vi "Performance Test.vi"() -> ()   [LabVIEW 2021]
uses:
  typedef/Topic Full Names.ctl
  <vilib>/Platform/TimedLoop/XDataNode/timing_clust.ctl
  <vilib>/Platform/TimedLoop/XDataNode/nitl_modes.ctl
  <vilib>/Platform/TimedLoop/XDataNode/wakeup.ctl
  1d7c6f29-a82a-4c55-90c2-8d5dc10d4cfc.vi
  17fd5a01-9941-4072-bead-c11bfc9bccae.vi
  ed299c19-1de2-4aef-bebd-b48bd10f6d98.vi
  968a0517-1209-4268-883c-89309fdc9691.vi
  d644dcab-1457-4dd0-b19b-55e0bc57f857.vi
  a6d30745-cc28-47f9-89da-0309ddd02839.vi
  ca39f006-b041-4da7-9f13-a82cb085cbb3.vi
  5bfc589c-c630-4e63-a8b4-f54732edfa77.vi
  394fcb2d-213c-4a5d-8836-742277111c33.vi
  47ad3e17-e753-4109-9264-7bc845309f70.vi
  34d71a64-62ff-4078-a387-3a58d5c35b2e.vi
  5417b091-9016-444e-b18d-e7968ccf46ca.vi
  17355536-f9ad-45df-8cdf-a653dafc3748.vi
  31a05237-38ce-4d36-92b2-ec91211d35c9.vi
  29b1b57c-db52-4db6-85d2-2783ba32f171.vi
  8285cac4-4baf-4ff9-aee7-9ff83ddf547c.vi
  d69192ad-9d02-4c06-9baa-091e86991072.vi
  801e2a67-ee41-44d4-a069-6c7db1e2d5be.vi
  84590647-50eb-4c0b-b77c-fbe9ef827284.vi
  20063719-1bf0-46dd-9a55-ff35ed26eb0a.vi
  38f10348-bd34-475b-a8eb-5ab5d485f78a.vi
  b3b3740b-c499-4e36-8042-ad8fb7248740.vi
  a2b9d25c-82f9-44a5-b179-014c788887ad.vi
  60e7bcfe-7ed0-4ed5-a910-62fb5c100d45.vi
  8a134818-91b4-4009-8209-aee668485e20.vi
  150ac17d-bb1a-4f1c-be46-9412ac39043d.vi
  1faeae08-4a57-41f3-9a76-3e5847141804.vi
  SubVIs/Get Path.vi
  SubVIs/Convert Error.vi
  1d7c6f29-a82a-4c55-90c2-8d5dc10d4cfc.vi/f164bb55-fadc-406a-97d8-e3295a396b46.vi
  SubVIs/Add Error.vi
  Refnum/BB from Refnum.vi
  Refnum/BB Writer to Refnum.vi
  <vilib>/CIF Foundation/CIF Utilities/File/File/File Not Found Error Update.vi
  17fd5a01-9941-4072-bead-c11bfc9bccae.vi/15451e88-64ef-462d-9cc0-58968935b893.vi
  Refnum/BB Reader to Refnum.vi
  Refnum/BB Writer from Refnum.vi
  Refnum/BB Reader from Refnum.vi
  5bfc589c-c630-4e63-a8b4-f54732edfa77.vi/f164bb55-fadc-406a-97d8-e3295a396b46.vi
  394fcb2d-213c-4a5d-8836-742277111c33.vi/15451e88-64ef-462d-9cc0-58968935b893.vi
  31a05237-38ce-4d36-92b2-ec91211d35c9.vi/f164bb55-fadc-406a-97d8-e3295a396b46.vi
  29b1b57c-db52-4db6-85d2-2783ba32f171.vi/15451e88-64ef-462d-9cc0-58968935b893.vi
  20063719-1bf0-46dd-9a55-ff35ed26eb0a.vi/3bd89bd1-b605-4b55-aa60-227046f12b11.vi
  38f10348-bd34-475b-a8eb-5ab5d485f78a.vi/bd005753-9160-49ee-ba23-7aa8055d86ff.vi
  Refnum/BB Raw Writer to Refnum.vi
  Refnum/BB Raw Reader to Refnum.vi
  Refnum/BB Raw Reader from Refnum.vi
  Refnum/BB Raw Writer from Refnum.vi
  <vilib>/Utility/error.llb/Trim Whitespace.vi
  SubVIs/Add Error Core.vi
  <vilib>/CIF Foundation/CIF Utilities/DataTypes/Utilities/Get Element Info of Variant.vi
  SubVIs/Get Type String.vi
  <vilib>/CIF Foundation/CIF Utilities/DataTypes/Utilities/Get JSON Descriptor of Variant.vi
  SubVIs/Convert Error Core.vi
  <vilib>/CIF Foundation/CIF Utilities/File/SubVIs/File Not Found Error Core.vi
  <vilib>/Platform/TimedLoop/XDataNode/XDataNode.xnode
  <vilib>/Platform/TimedLoop/XDataNode/XDNodeRunTimeDep.lvlib
  Iceoryx.lvlib
panel:
  out "avg read raw large array":dbl
  out "max read raw large array":dbl
  out "avg read large array":dbl
  out "max read large array":dbl
  out "avg write double":dbl
  out "max write double":dbl
  out "avg read double no writer":dbl
  out "max read double no writer":dbl
  in  "stop":bool
  out "avg read double":dbl
  out "max read double":dbl
  out "pass":bool
  out "error out":errorcluster
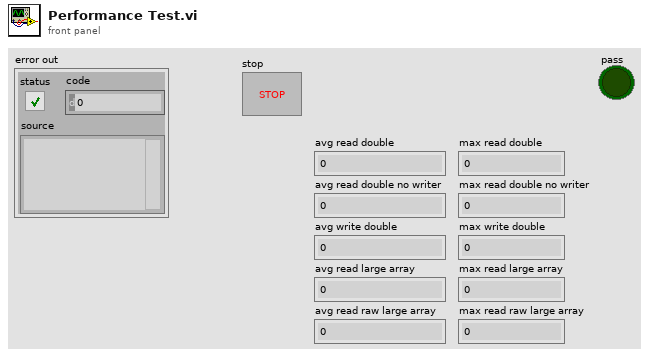
[diagram p1: front panel]
types:
  T1 = typedef "Iceoryx.lvlib/Topic Full Names.ctl" = cluster{"BlackBoard":string, "Topic":string, "Type Override":string}
  T2 = typedef "XDNodeRunTimeDep.lvlib/timing_clust.ctl" = cluster{"Expected End [f-1]":u64, "Actual End [f-1]":u64, "Finished Late? [f-1]":bool, "Expected End [i-1]":u64, "Actual End [i-1]":u64, "Finished Late? [i-1]":bool, "Expected Start [i]":u64, "Actual Start [i]":u64, "Expected Start [f]":u64, "Actual Start [f]":u64, "Source Name":string, "Structure Name":string, "Period":i64, "Deadline":i64, "Offset":i64, "Start":i64, "Priority":i32, "Timeout":i32, "Mode":T3, "Wakeup Reason":T4, "Error":errorcluster, "Source Type":string, "Secondary Source Type":string, "Global End Time":u64, "Global Start Time":u64, "Frame Duration":u64, "Iteration Duration":u64, "Assigned CPU":i32, "I/O Scan Engine Mode":u32}
  T3 = typedef "XDNodeRunTimeDep.lvlib/nitl_modes.ctl" = enum32{"No Change", "Process missed periods, maintain original phase", "Discard missed periods, maintain original phase", "Process missed periods, ignore original phase", "Discard missed periods, ignore original phase"}
  T4 = typedef "XDNodeRunTimeDep.lvlib/wakeup.ctl" = enum32{"Normal", "Aborted", "Asynchronous wakeup", "Timing source error", "Timed loop error", "Timeout"}
  T5 = typedef "Iceoryx.lvlib/BB Refnum.ctl" = cluster{"refnum":u64, "BB":enum8{"bb"}}
  T6 = typedef "Iceoryx.lvlib/BB Writer Refnum.ctl" = cluster{"refnum":u64, "BB Writer":enum8{"bb_writer"}}
  T7 = typedef "Iceoryx.lvlib/BB Reader Refnum.ctl" = cluster{"refnum":u64, "BB Reader":enum8{"bb_reader"}}
  T8 = typedef "Iceoryx.lvlib/BB Raw Writer Refnum.ctl" = cluster{"refnum":u64, "BB Raw Writer":enum8{"bb_raw_writer"}}
  T9 = typedef "Iceoryx.lvlib/BB Raw Reader Refnum.ctl" = cluster{"refnum":u64, "BB Raw Reader":enum8{"bb_raw_reader"}}
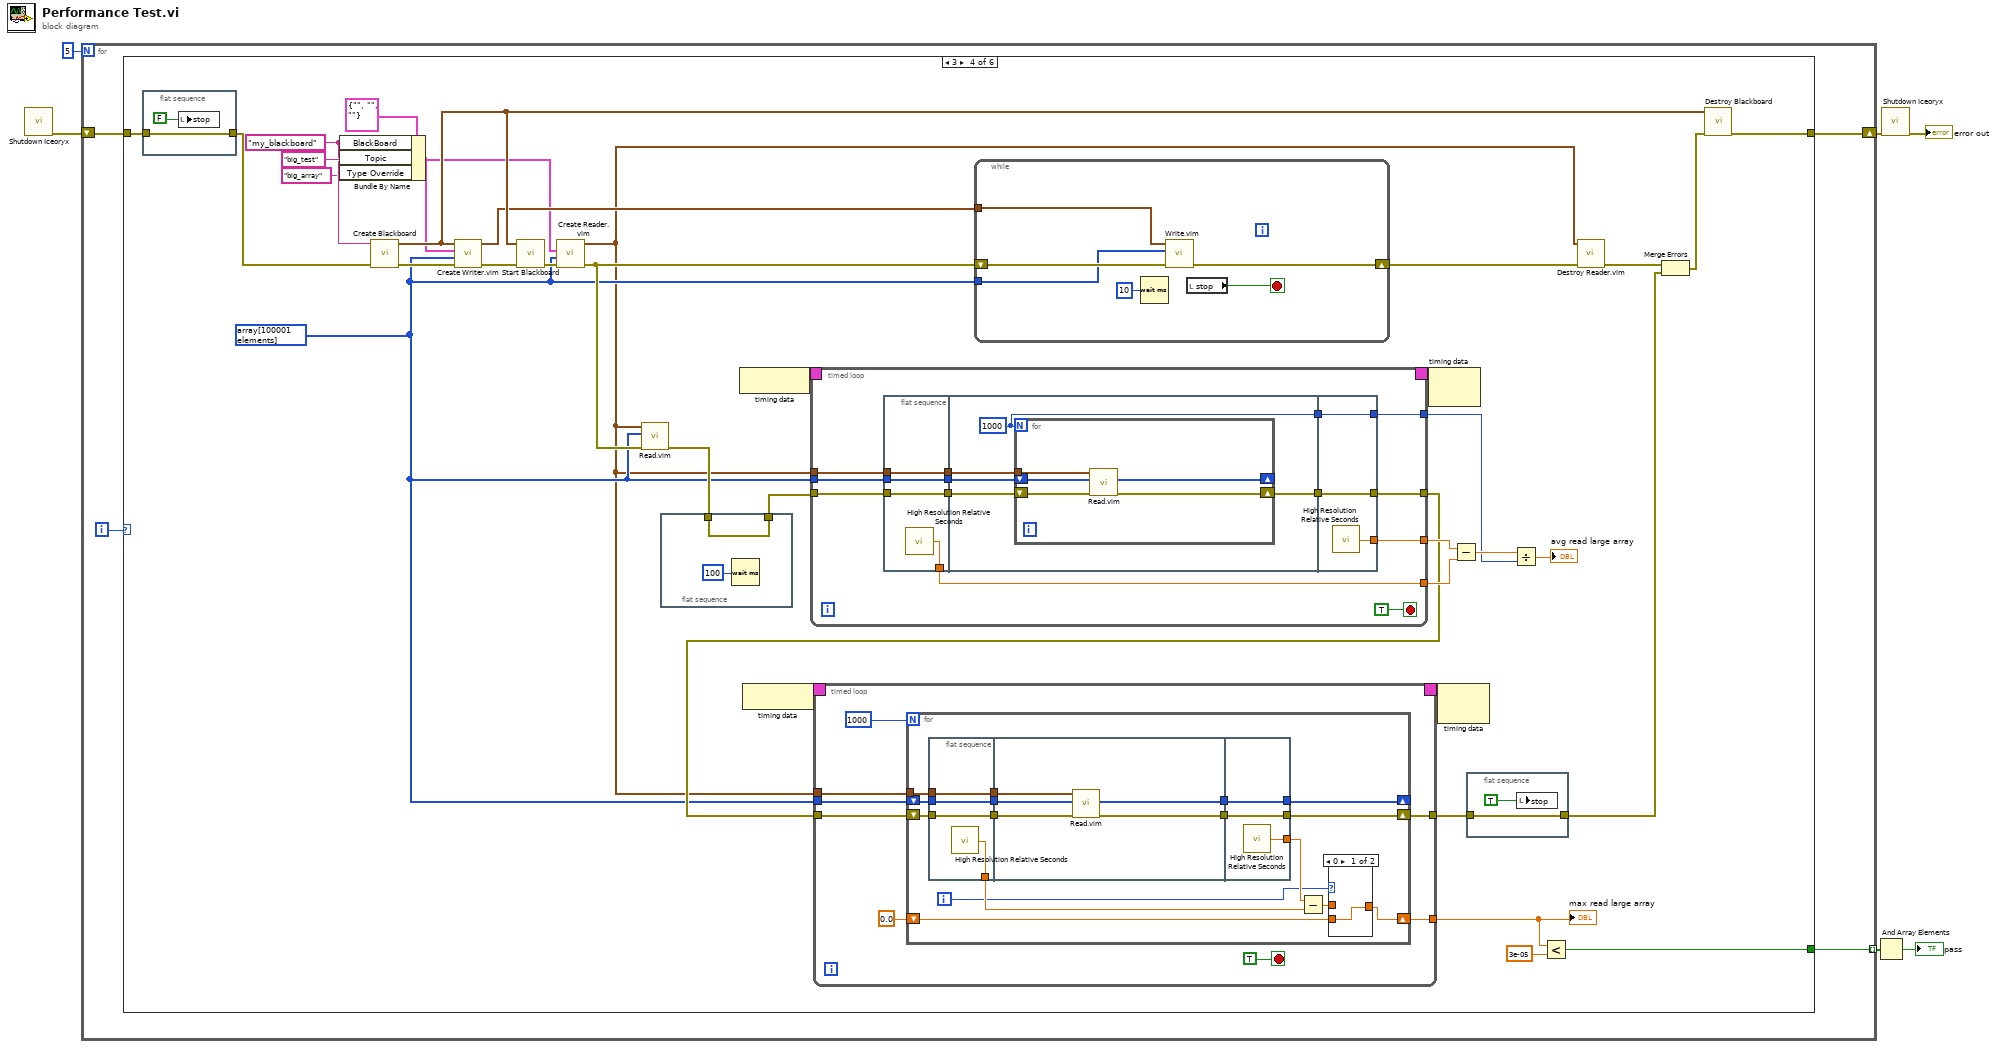
[diagram p0: block diagram]
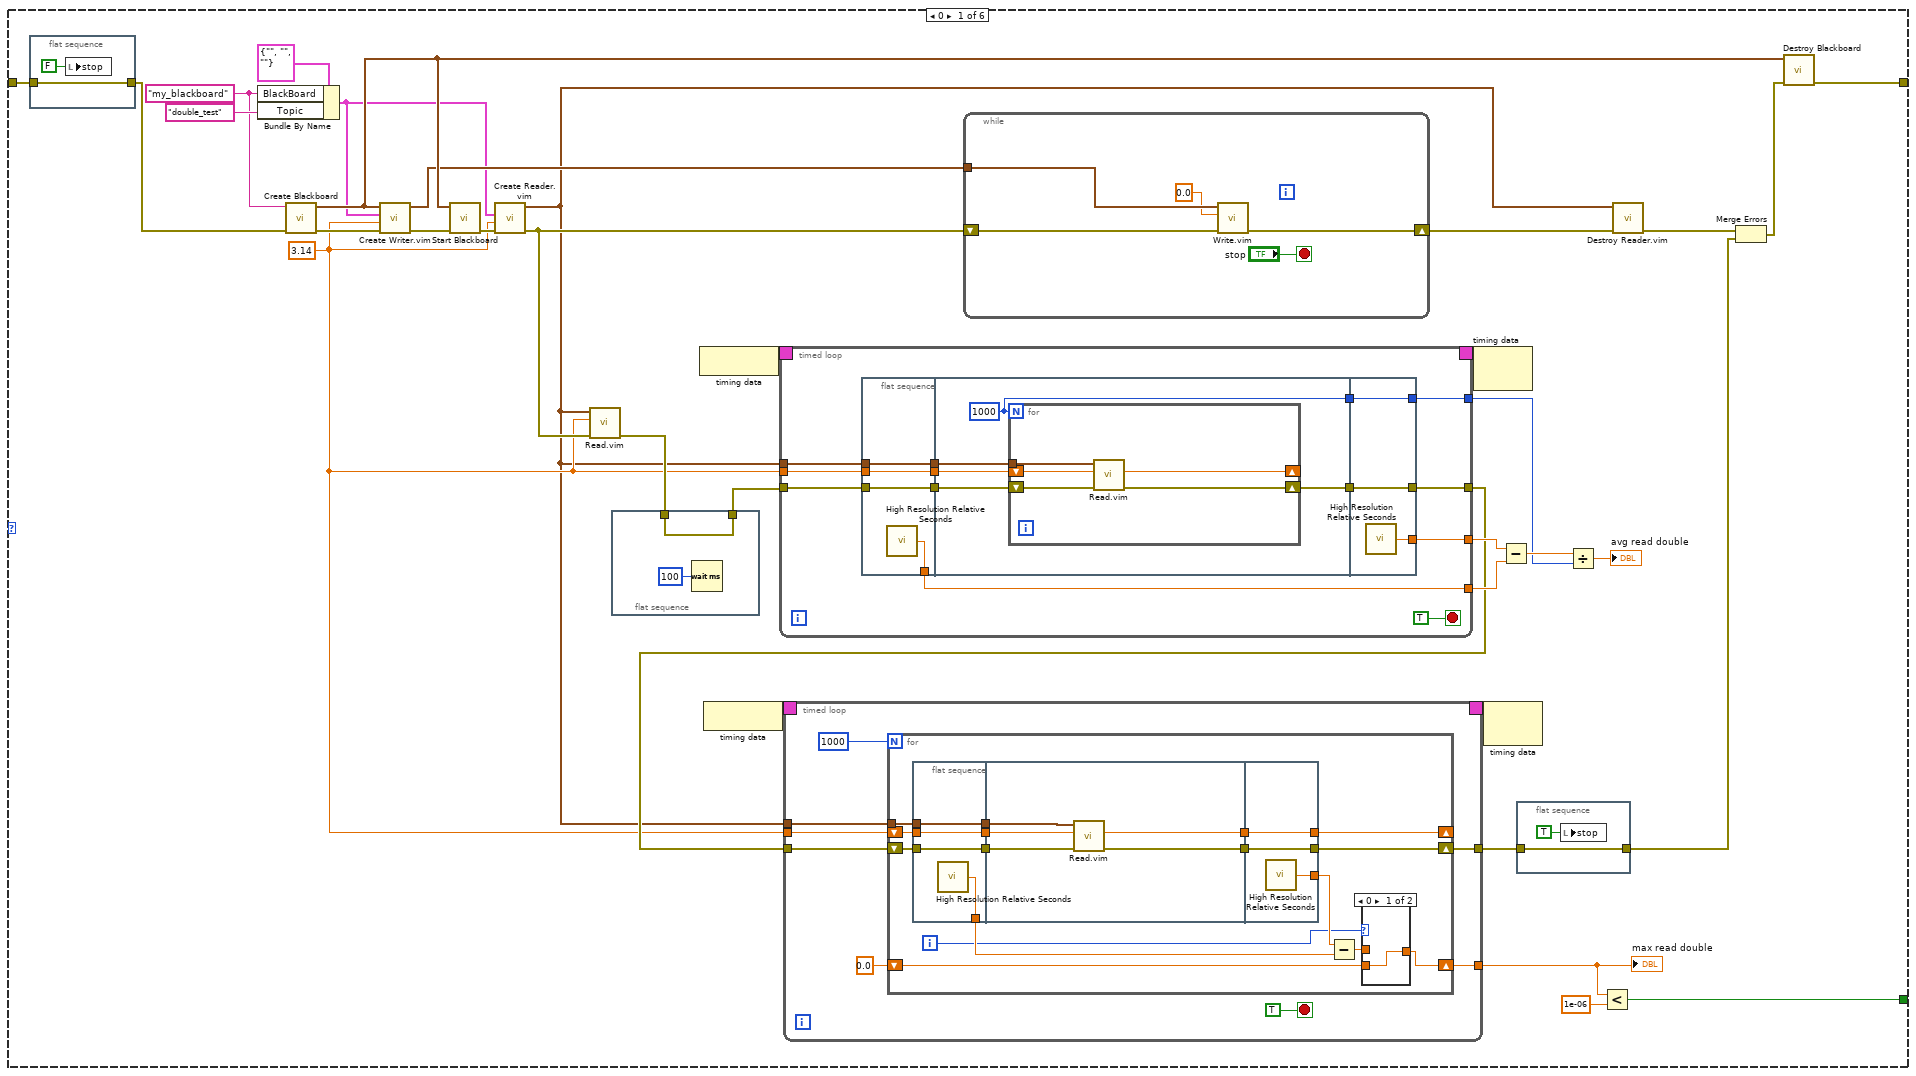
[diagram p2: hidden frame]
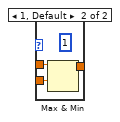
[diagram p3: hidden frame]
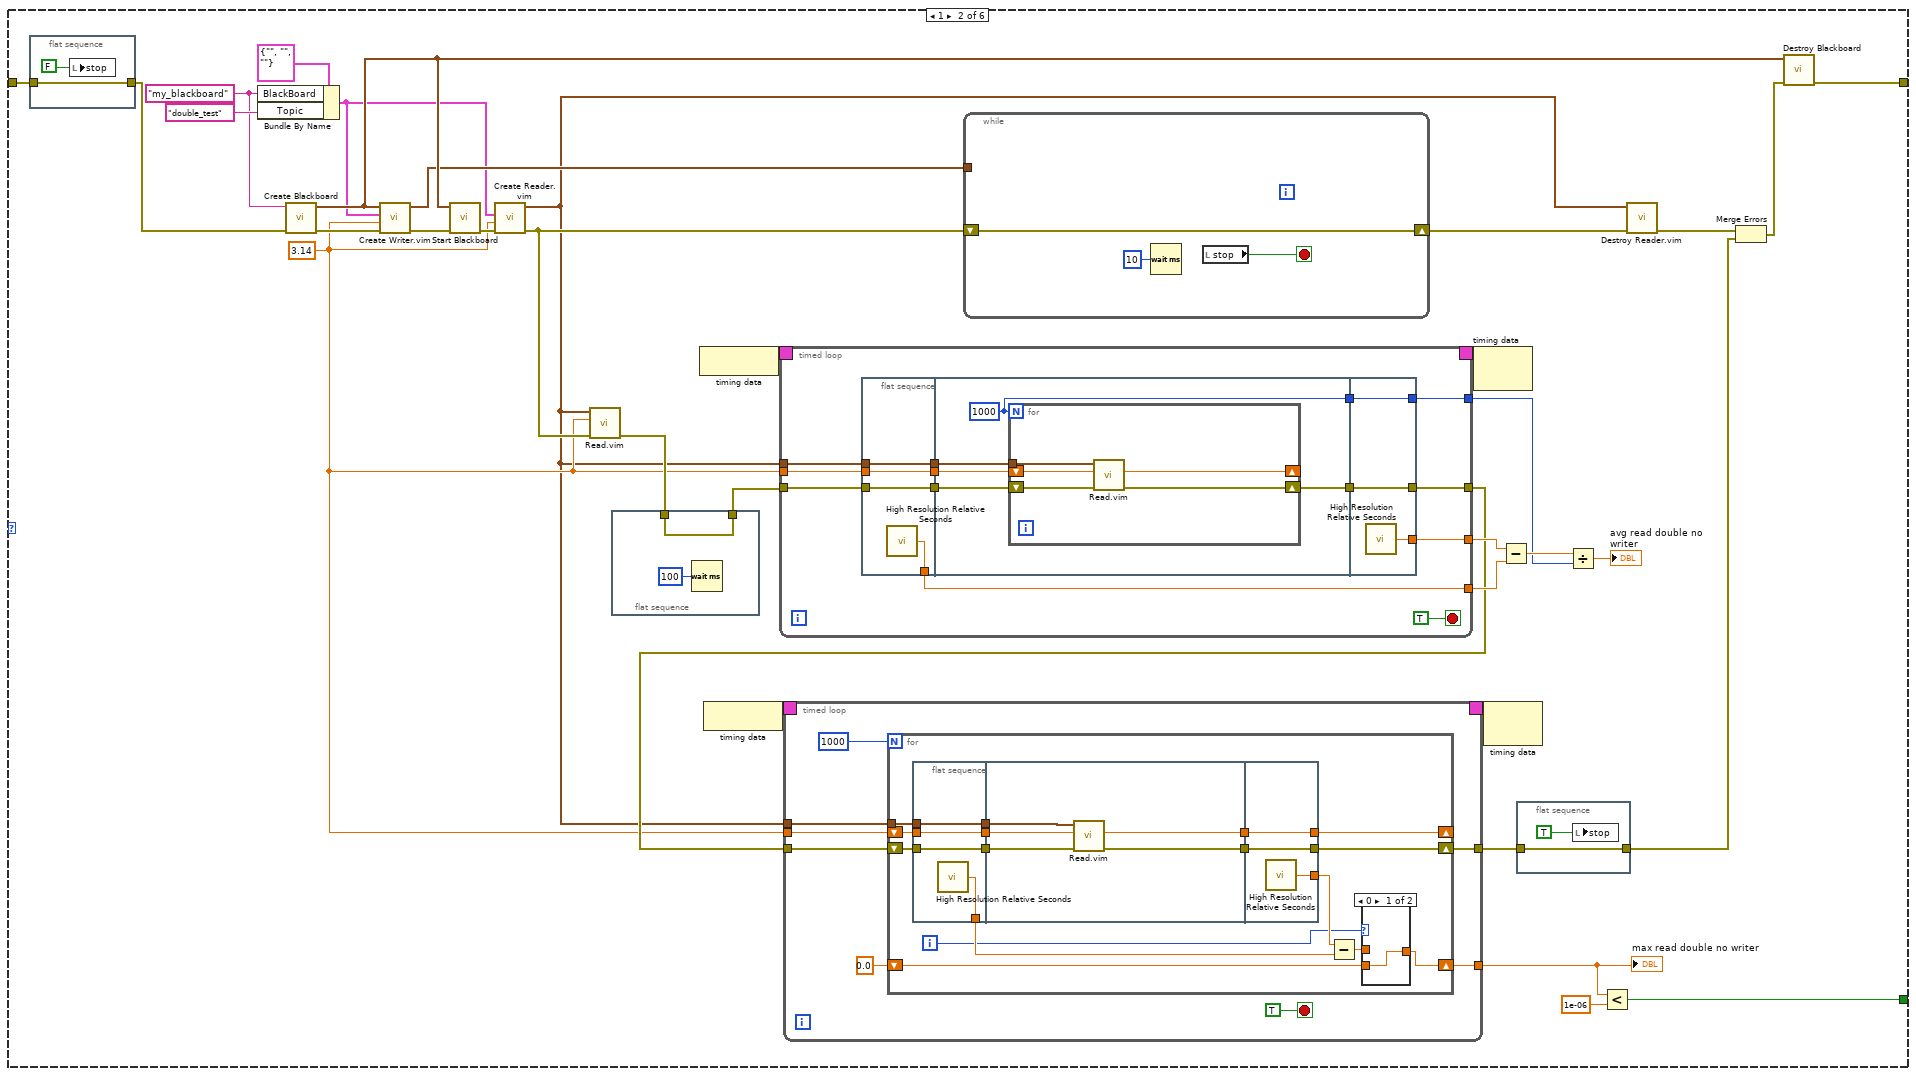
[diagram p4: hidden frame]
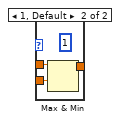
[diagram p5: hidden frame]
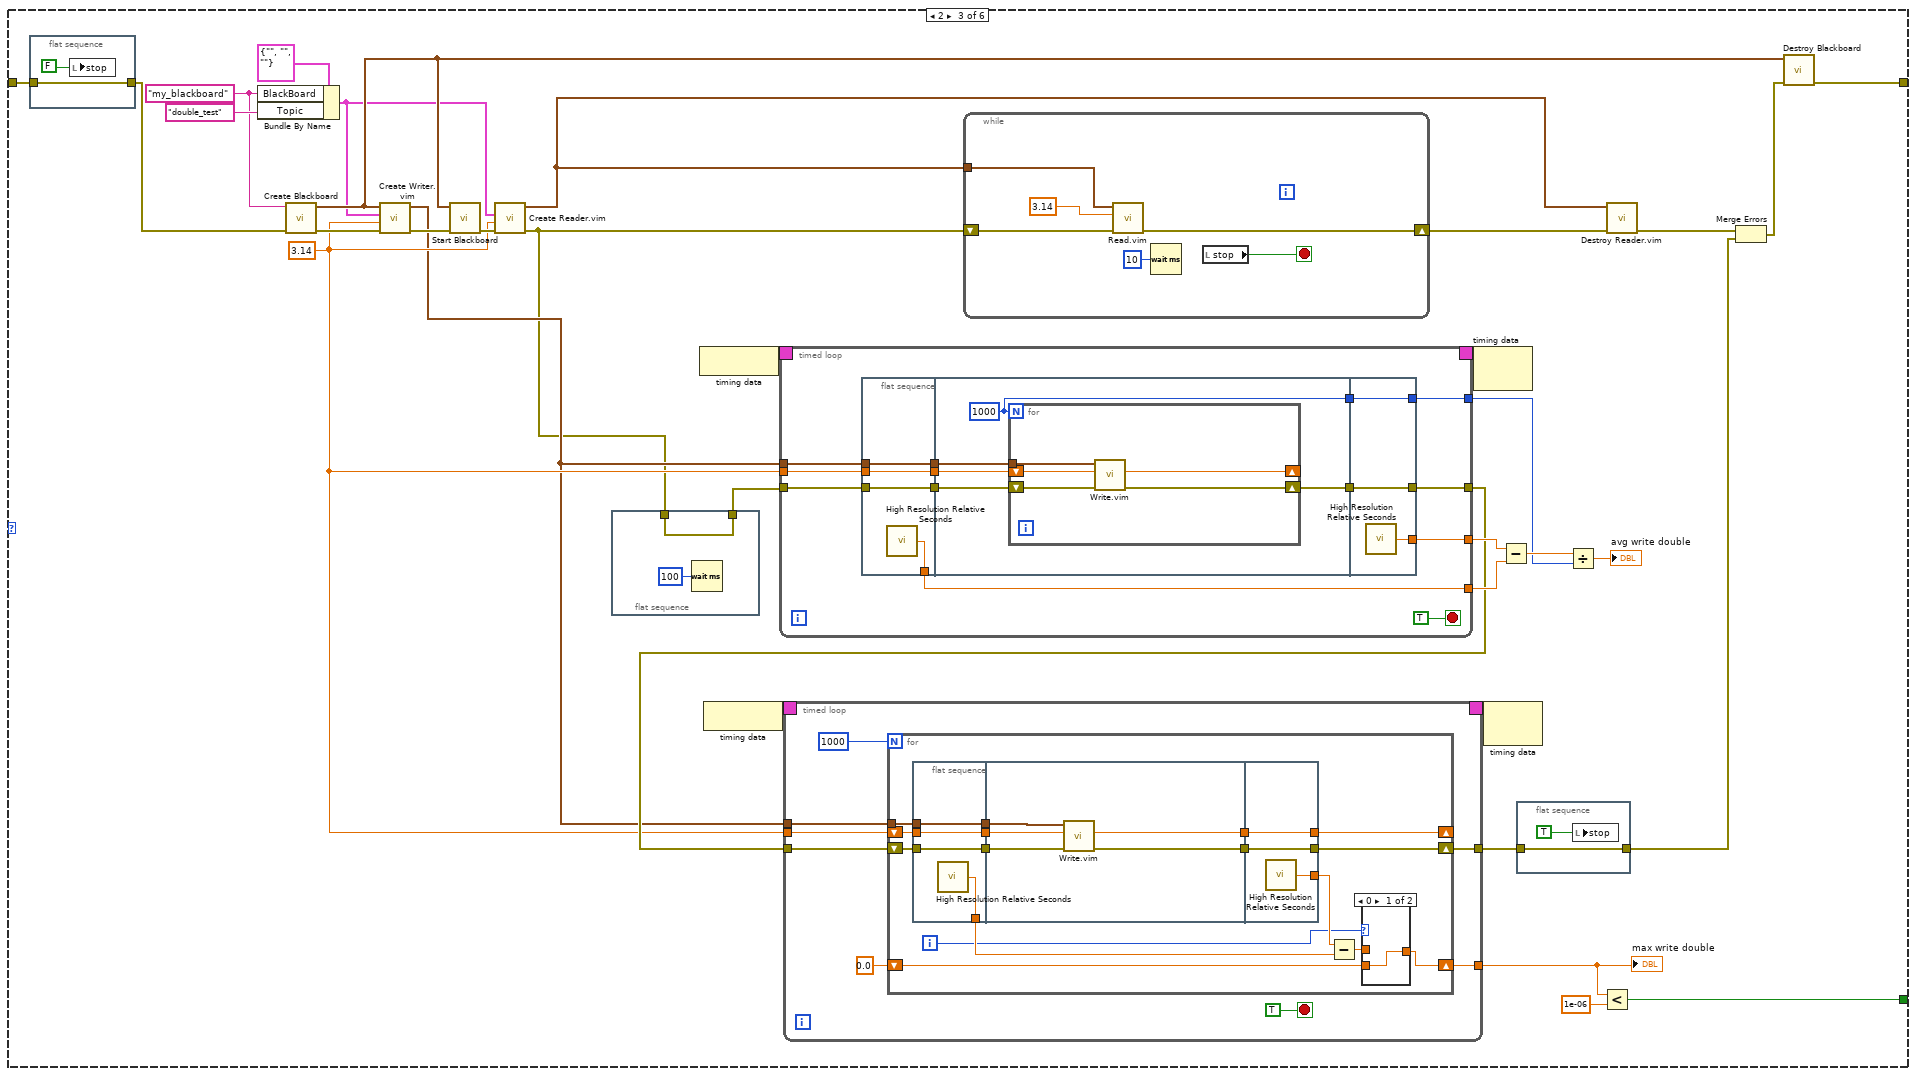
[diagram p6: hidden frame]
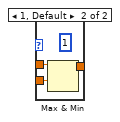
[diagram p7: hidden frame]
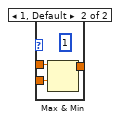
[diagram p8: hidden frame]
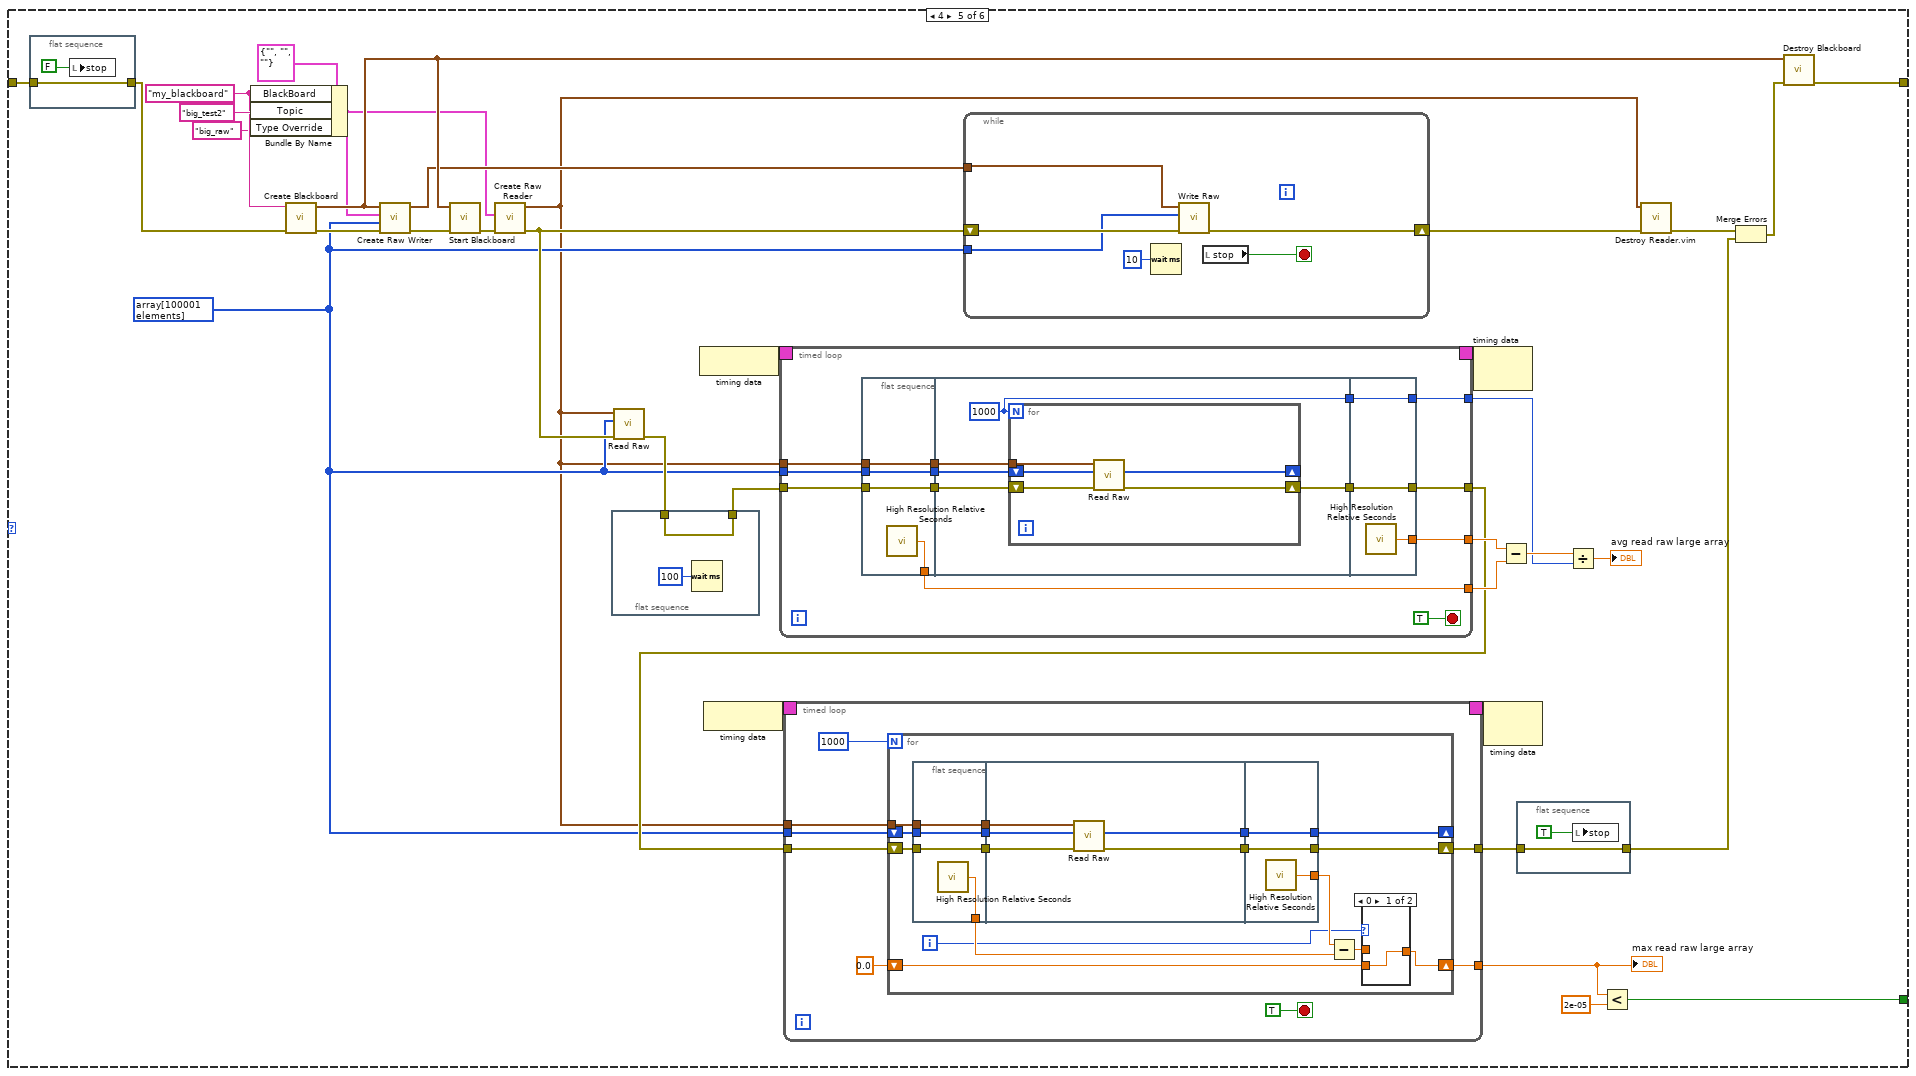
[diagram p9: hidden frame]
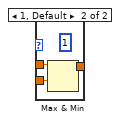
[diagram p10: hidden frame]
diagram:
  n1 = call "Shutdown Iceoryx.vi"() -> ("error out"=w4:errorcluster)  [unwired: 11 in]
  n2 = for {
    N: 5 -> [_]
    tunnel: [w10] -> w2 mode=indexing
    shift-right: [w9] -> w6
    shift-left: w4 -> [w8]
    i -> [w7]
    n3 = case shown="3" w7 {
      tunnel: [w31 w155 w276 w402 w528 _] -> w10
      tunnel: [w26 w150 w271 w397 w523 w633] -> w9
      tunnel: w8 -> [w15 w139 w263 w387 w515 w633]
      frame 0 {
        w19 = "my_blackboard" ("Blackboard name")
        w18 = 3.14 ("Data")
        n4 = flat-sequence {
          tunnel: w15 -> [w52]
          tunnel: [w52] -> w14
          frame #0 {
            n5 = local write "stop"(FALSE ("stop")) -> ()
          }
        }
        n6 = Bundle By Name(cluster=T1 {"BlackBoard"="", "Topic"="", "Type Override"=""} ("Topic Full Names"), "BlackBoard"=w19, "Topic"="double_test" ("topic")) -> (w20:T1)
        n7 = call "Create Blackboard.vi"("error in (no error)"=w14, "Blackboard name"=w19) -> ("error out"=w30:errorcluster, "Blackboard Reference"=w28:T5)  [unwired: 8 in]
        n8 = call "Create Writer.vim"("error in (no error)"=w30, "Data"=w18, "Topic Name"=w20, "BlackBoard Reference"=w28) -> ("error out"=w29:errorcluster, "Writer Reference"=w25:T6)  [unwired: 5 in, 1 out]
        n9 = call "Start Blackboard.vi"("error in (no error)"=w29, "Blackboard Reference"=w28) -> ("error out"=w27:errorcluster)  [unwired: 9 in]
        n10 = call "Create Reader.vim"("error in (no error)"=w27, "Data Type"=w18, "Topic Name"=w20) -> ("error out"=w24:errorcluster, "Reader Reference"=w11:T7)  [unwired: 6 in, 1 out]
        n11 = call "Read.vim"("error in (no error)"=w24, "Data In"=w18, "Reader Reference"=w11) -> ("error out"=w23:errorcluster)  [unwired: 6 in, 2 out]
        n12 = flat-sequence {
          tunnel: w23 -> [w56]
          tunnel: [w56] -> w33
          frame #0 {
            n13 = Wait (ms)(milliseconds to wait=u32 100) -> ()  [unwired: 1 out]
          }
        }
        n14 = node-c288() -> (w45:T2)
        n15 = node-c288() -> (w43:T2)
        n16 = timed-loop {
          timing: w45 -> [_]
          timing-out: [_] -> w44
          tunnel: w11 -> [w103]
          tunnel: w33 -> [w113]
          tunnel: [w110] -> w37
          tunnel: [w108] -> w41
          tunnel: [w107] -> w40
          tunnel: [w106] -> w38
          tunnel: w18 -> [w101]
          stop <- TRUE stop-if-true
          n17 = flat-sequence {
            tunnel: w113 -> [w117]
            tunnel: [w117] -> w111
            tunnel: [w116] -> w107
            tunnel: [w115] -> w104
            tunnel: w103 -> [w115]
            tunnel: [w114] -> w102
            tunnel: w101 -> [w114]
            tunnel: w111 -> [w122]
            tunnel: [w121] -> w109
            tunnel: [w120] -> w105
            tunnel: w104 -> [w119]
            tunnel: w102 -> [w118]
            tunnel: [w130] -> w110
            tunnel: w109 -> [w130]
            tunnel: [w129] -> w108
            tunnel: [w128] -> w106
            tunnel: w105 -> [w128]
            frame #0 {
              n18 = call <vilib>:"High Resolution Relative Seconds.vi"() -> ("relative seconds"=w116:dbl)
            }
            frame #1 {
              w120 = 1000
              n19 = for {
                N: w120 -> [_]
                shift-right: [w124] -> _
                shift-left: w118 -> [w123]
                shift-right: [w125] -> w121
                shift-left: w122 -> [w126]
                tunnel: w119 -> [w127]
                n20 = call "Read.vim"("error in (no error)"=w126, "Data In"=w123, "Reader Reference"=w127) -> ("error out"=w125:errorcluster, "Data Out"=w124:dbl)  [unwired: 6 in, 1 out]
              }
            }
            frame #2 {
              n21 = call <vilib>:"High Resolution Relative Seconds.vi"() -> ("relative seconds"=w129:dbl)
            }
          }
        }
        n22 = timed-loop {
          timing: w43 -> [_]
          timing-out: [_] -> w42
          tunnel: w37 -> [w64]
          tunnel: [w62] -> w32
          tunnel: [w59] -> w35
          tunnel: w18 -> [w58]
          tunnel: w11 -> [w57]
          stop <- TRUE stop-if-true
          n23 = for {
            N: 1000 -> [_]
            shift-right: [w75] -> _
            shift-left: w58 -> [w77]
            shift-right: [w74] -> w62
            shift-left: w64 -> [w76]
            shift-right: [w69] -> w59
            shift-left: 0.0 -> [w70]
            tunnel: w57 -> [w65]
            i -> [w68]
            n24 = flat-sequence {
              tunnel: w76 -> [w87]
              tunnel: w77 -> [w88]
              tunnel: [w88] -> w80
              tunnel: [w87] -> w79
              tunnel: [w86] -> w72
              tunnel: [w85] -> w66
              tunnel: w65 -> [w85]
              tunnel: w80 -> [w89]
              tunnel: w79 -> [w93]
              tunnel: [w91] -> w78
              tunnel: [w90] -> w67
              tunnel: w66 -> [w92]
              tunnel: [w96] -> w75
              tunnel: w78 -> [w96]
              tunnel: [w95] -> w74
              tunnel: [w94] -> w73
              tunnel: w67 -> [w95]
              frame #0 {
                n25 = call <vilib>:"High Resolution Relative Seconds.vi"() -> ("relative seconds"=w86:dbl)
              }
              frame #1 {
                n26 = call "Read.vim"("error in (no error)"=w93, "Data In"=w89, "Reader Reference"=w92) -> ("error out"=w90:errorcluster, "Data Out"=w91:dbl)  [unwired: 6 in, 1 out]
              }
              frame #2 {
                n27 = call <vilib>:"High Resolution Relative Seconds.vi"() -> ("relative seconds"=w94:dbl)
              }
            }
            n28 = Subtract(x=w73, y=w72) -> (x-y=w71:dbl)
            n29 = case shown="0" w68 {
              tunnel: w71 -> [_ w84]
              tunnel: w70 -> [w81 w83]
              tunnel: [w81 w82] -> w69
              frame 0 {
              }
              frame 1, Default {
                (unwired) u32 1 ("milliseconds to wait")
                n30 = Max & Min(x=w84, y=w83) -> (max(x,y)=w82:dbl)  [unwired: 1 out]
              }
            }
          }
        }
        "max read double" <- w35
        n31 = while {
          shift-right: [w47] -> w13
          shift-left: w24 -> [w48]
          tunnel: w25 -> [w49]
          stop <- "stop" stop-if-true
          n32 = call "Write.vim"("error in (no error)"=w48, "Data In"=0.0, "Writer Reference"=w49) -> ("error out"=w47:errorcluster)  [unwired: 7 in, 1 out]
        }
        n33 = node-c288(w44) -> ()  [unwired: 1 out]
        n34 = node-c288(w42) -> ()  [unwired: 1 out]
        n35 = Subtract(x=w41, y=w40) -> (x-y=w39:dbl)
        n36 = flat-sequence {
          tunnel: w32 -> [w54]
          tunnel: [w54] -> w17
          frame #0 {
            n37 = local write "stop"(TRUE ("stop")) -> ()
          }
        }
        n38 = Divide(x=w39, y=w38) -> (x/y=→"avg read double":dbl)
        n39 = Less?(x=w35, y=1e-06) -> (x < y?=w31:bool)
        n40 = call "Destroy Reader.vim"("error in (no error)"=w13, "Reader Reference"=w11) -> ("error out"=w12:errorcluster)  [unwired: 9 in]
        n41 = Merge Errors(w12, w17) -> (w16:errorcluster)
        n42 = call "Destroy Blackboard.vi"("error in (no error)"=w16, "Blackboard Reference"=w28) -> ("error out"=w26:errorcluster)  [unwired: 8 in, 1 out]
      }
      frame 1 {
        w143 = "my_blackboard" ("Blackboard name")
        w142 = 3.14 ("Data")
        n43 = flat-sequence {
          tunnel: w139 -> [w174]
          tunnel: [w174] -> w138
          frame #0 {
            n44 = local write "stop"(FALSE ("stop")) -> ()
          }
        }
        n45 = Bundle By Name(cluster=T1 {"BlackBoard"="", "Topic"="", "Type Override"=""} ("Topic Full Names"), "BlackBoard"=w143, "Topic"="double_test" ("topic")) -> (w144:T1)
        n46 = call "Create Blackboard.vi"("error in (no error)"=w138, "Blackboard name"=w143) -> ("error out"=w154:errorcluster, "Blackboard Reference"=w152:T5)  [unwired: 8 in]
        n47 = call "Create Writer.vim"("error in (no error)"=w154, "Data"=w142, "Topic Name"=w144, "BlackBoard Reference"=w152) -> ("error out"=w153:errorcluster, "Writer Reference"=w149:T6)  [unwired: 5 in, 1 out]
        n48 = call "Start Blackboard.vi"("error in (no error)"=w153, "Blackboard Reference"=w152) -> ("error out"=w151:errorcluster)  [unwired: 9 in]
        n49 = call "Create Reader.vim"("error in (no error)"=w151, "Data Type"=w142, "Topic Name"=w144) -> ("error out"=w148:errorcluster, "Reader Reference"=w135:T7)  [unwired: 6 in, 1 out]
        n50 = call "Read.vim"("error in (no error)"=w148, "Data In"=w142, "Reader Reference"=w135) -> ("error out"=w147:errorcluster)  [unwired: 6 in, 2 out]
        n51 = flat-sequence {
          tunnel: w147 -> [w178]
          tunnel: [w178] -> w157
          frame #0 {
            n52 = Wait (ms)(milliseconds to wait=u32 100) -> ()  [unwired: 1 out]
          }
        }
        n53 = node-c288() -> (w169:T2)
        n54 = node-c288() -> (w167:T2)
        n55 = timed-loop {
          timing: w169 -> [_]
          timing-out: [_] -> w168
          tunnel: w135 -> [w225]
          tunnel: w157 -> [w235]
          tunnel: [w232] -> w161
          tunnel: [w230] -> w165
          tunnel: [w229] -> w164
          tunnel: [w228] -> w162
          tunnel: w142 -> [w223]
          stop <- TRUE stop-if-true
          n56 = flat-sequence {
            tunnel: w235 -> [w239]
            tunnel: [w239] -> w233
            tunnel: [w238] -> w229
            tunnel: [w237] -> w226
            tunnel: w225 -> [w237]
            tunnel: [w236] -> w224
            tunnel: w223 -> [w236]
            tunnel: w233 -> [w244]
            tunnel: [w243] -> w231
            tunnel: [w242] -> w227
            tunnel: w226 -> [w241]
            tunnel: w224 -> [w240]
            tunnel: [w252] -> w232
            tunnel: w231 -> [w252]
            tunnel: [w251] -> w230
            tunnel: [w250] -> w228
            tunnel: w227 -> [w250]
            frame #0 {
              n57 = call <vilib>:"High Resolution Relative Seconds.vi"() -> ("relative seconds"=w238:dbl)
            }
            frame #1 {
              w242 = 1000
              n58 = for {
                N: w242 -> [_]
                shift-right: [w246] -> _
                shift-left: w240 -> [w245]
                shift-right: [w247] -> w243
                shift-left: w244 -> [w248]
                tunnel: w241 -> [w249]
                n59 = call "Read.vim"("error in (no error)"=w248, "Data In"=w245, "Reader Reference"=w249) -> ("error out"=w247:errorcluster, "Data Out"=w246:dbl)  [unwired: 6 in, 1 out]
              }
            }
            frame #2 {
              n60 = call <vilib>:"High Resolution Relative Seconds.vi"() -> ("relative seconds"=w251:dbl)
            }
          }
        }
        n61 = timed-loop {
          timing: w167 -> [_]
          timing-out: [_] -> w166
          tunnel: w161 -> [w186]
          tunnel: [w184] -> w156
          tunnel: [w181] -> w159
          tunnel: w142 -> [w180]
          tunnel: w135 -> [w179]
          stop <- TRUE stop-if-true
          n62 = for {
            N: 1000 -> [_]
            shift-right: [w197] -> _
            shift-left: w180 -> [w199]
            shift-right: [w196] -> w184
            shift-left: w186 -> [w198]
            shift-right: [w191] -> w181
            shift-left: 0.0 -> [w192]
            tunnel: w179 -> [w187]
            i -> [w190]
            n63 = flat-sequence {
              tunnel: w198 -> [w209]
              tunnel: w199 -> [w210]
              tunnel: [w210] -> w202
              tunnel: [w209] -> w201
              tunnel: [w208] -> w194
              tunnel: [w207] -> w188
              tunnel: w187 -> [w207]
              tunnel: w202 -> [w211]
              tunnel: w201 -> [w215]
              tunnel: [w213] -> w200
              tunnel: [w212] -> w189
              tunnel: w188 -> [w214]
              tunnel: [w218] -> w197
              tunnel: w200 -> [w218]
              tunnel: [w217] -> w196
              tunnel: [w216] -> w195
              tunnel: w189 -> [w217]
              frame #0 {
                n64 = call <vilib>:"High Resolution Relative Seconds.vi"() -> ("relative seconds"=w208:dbl)
              }
              frame #1 {
                n65 = call "Read.vim"("error in (no error)"=w215, "Data In"=w211, "Reader Reference"=w214) -> ("error out"=w212:errorcluster, "Data Out"=w213:dbl)  [unwired: 6 in, 1 out]
              }
              frame #2 {
                n66 = call <vilib>:"High Resolution Relative Seconds.vi"() -> ("relative seconds"=w216:dbl)
              }
            }
            n67 = Subtract(x=w195, y=w194) -> (x-y=w193:dbl)
            n68 = case shown="0" w190 {
              tunnel: w193 -> [_ w206]
              tunnel: w192 -> [w203 w205]
              tunnel: [w203 w204] -> w191
              frame 0 {
              }
              frame 1, Default {
                (unwired) u32 1 ("milliseconds to wait")
                n69 = Max & Min(x=w206, y=w205) -> (max(x,y)=w204:dbl)  [unwired: 1 out]
              }
            }
          }
        }
        "max read double no writer" <- w159
        n70 = while {
          shift-right: [w171] -> w137
          shift-left: w148 -> [w171]
          tunnel: w149 -> [_]
          stop <- w170 stop-if-true
          n71 = Wait (ms)(milliseconds to wait=u32 10) -> ()  [unwired: 1 out]
          n72 = local read "stop"() -> (w170:bool)
        }
        n73 = node-c288(w168) -> ()  [unwired: 1 out]
        n74 = node-c288(w166) -> ()  [unwired: 1 out]
        n75 = Subtract(x=w165, y=w164) -> (x-y=w163:dbl)
        n76 = flat-sequence {
          tunnel: w156 -> [w176]
          tunnel: [w176] -> w141
          frame #0 {
            n77 = local write "stop"(TRUE ("stop")) -> ()
          }
        }
        n78 = Divide(x=w163, y=w162) -> (x/y=→"avg read double no writer":dbl)
        n79 = Less?(x=w159, y=1e-06) -> (x < y?=w155:bool)
        n80 = call "Destroy Reader.vim"("error in (no error)"=w137, "Reader Reference"=w135) -> ("error out"=w136:errorcluster)  [unwired: 9 in]
        n81 = Merge Errors(w136, w141) -> (w140:errorcluster)
        n82 = call "Destroy Blackboard.vi"("error in (no error)"=w140, "Blackboard Reference"=w152) -> ("error out"=w150:errorcluster)  [unwired: 8 in, 1 out]
      }
      frame 2 {
        w267 = "my_blackboard" ("Blackboard name")
        w266 = 3.14 ("Data")
        n83 = flat-sequence {
          tunnel: w263 -> [w298]
          tunnel: [w298] -> w262
          frame #0 {
            n84 = local write "stop"(FALSE ("stop")) -> ()
          }
        }
        n85 = Bundle By Name(cluster=T1 {"BlackBoard"="", "Topic"="", "Type Override"=""} ("Topic Full Names"), "BlackBoard"=w267, "Topic"="double_test" ("topic")) -> (w268:T1)
        n86 = call "Create Blackboard.vi"("error in (no error)"=w262, "Blackboard name"=w267) -> ("error out"=w275:errorcluster, "Blackboard Reference"=w273:T5)  [unwired: 8 in]
        n87 = call "Create Writer.vim"("error in (no error)"=w275, "Data"=w266, "Topic Name"=w268, "BlackBoard Reference"=w273) -> ("error out"=w274:errorcluster, "Writer Reference"=w261:T6)  [unwired: 5 in, 1 out]
        n88 = call "Start Blackboard.vi"("error in (no error)"=w274, "Blackboard Reference"=w273) -> ("error out"=w272:errorcluster)  [unwired: 9 in]
        n89 = call "Create Reader.vim"("error in (no error)"=w272, "Data Type"=w266, "Topic Name"=w268) -> ("error out"=w260:errorcluster, "Reader Reference"=w257:T7)  [unwired: 6 in, 1 out]
        n90 = flat-sequence {
          tunnel: w260 -> [w302]
          tunnel: [w302] -> w278
          frame #0 {
            n91 = Wait (ms)(milliseconds to wait=u32 100) -> ()  [unwired: 1 out]
          }
        }
        n92 = node-c288() -> (w290:T2)
        n93 = node-c288() -> (w288:T2)
        n94 = timed-loop {
          timing: w290 -> [_]
          timing-out: [_] -> w289
          tunnel: w261 -> [w349]
          tunnel: w278 -> [w359]
          tunnel: [w356] -> w282
          tunnel: [w354] -> w286
          tunnel: [w353] -> w285
          tunnel: [w352] -> w283
          tunnel: w266 -> [w347]
          stop <- TRUE stop-if-true
          n95 = flat-sequence {
            tunnel: w359 -> [w363]
            tunnel: [w363] -> w357
            tunnel: [w362] -> w353
            tunnel: [w361] -> w350
            tunnel: w349 -> [w361]
            tunnel: [w360] -> w348
            tunnel: w347 -> [w360]
            tunnel: w357 -> [w368]
            tunnel: [w367] -> w355
            tunnel: [w366] -> w351
            tunnel: w350 -> [w365]
            tunnel: w348 -> [w364]
            tunnel: [w376] -> w356
            tunnel: w355 -> [w376]
            tunnel: [w375] -> w354
            tunnel: [w374] -> w352
            tunnel: w351 -> [w374]
            frame #0 {
              n96 = call <vilib>:"High Resolution Relative Seconds.vi"() -> ("relative seconds"=w362:dbl)
            }
            frame #1 {
              w366 = 1000
              n97 = for {
                N: w366 -> [_]
                shift-right: [w369] -> _
                shift-left: w364 -> [w371]
                shift-right: [w370] -> w367
                shift-left: w368 -> [w373]
                tunnel: w365 -> [w372]
                n98 = call "Write.vim"("error in (no error)"=w373, "Data In"=w371, "Writer Reference"=w372) -> ("error out"=w370:errorcluster, "Data Out"=w369:dbl)  [unwired: 7 in]
              }
            }
            frame #2 {
              n99 = call <vilib>:"High Resolution Relative Seconds.vi"() -> ("relative seconds"=w375:dbl)
            }
          }
        }
        n100 = timed-loop {
          timing: w288 -> [_]
          timing-out: [_] -> w287
          tunnel: w282 -> [w310]
          tunnel: [w308] -> w277
          tunnel: [w305] -> w280
          tunnel: w266 -> [w304]
          tunnel: w261 -> [w303]
          stop <- TRUE stop-if-true
          n101 = for {
            N: 1000 -> [_]
            shift-right: [w321] -> _
            shift-left: w304 -> [w323]
            shift-right: [w320] -> w308
            shift-left: w310 -> [w322]
            shift-right: [w315] -> w305
            shift-left: 0.0 -> [w316]
            tunnel: w303 -> [w311]
            i -> [w314]
            n102 = flat-sequence {
              tunnel: w322 -> [w333]
              tunnel: w323 -> [w334]
              tunnel: [w334] -> w326
              tunnel: [w333] -> w325
              tunnel: [w332] -> w318
              tunnel: [w331] -> w312
              tunnel: w311 -> [w331]
              tunnel: w326 -> [w336]
              tunnel: w325 -> [w339]
              tunnel: [w337] -> w324
              tunnel: [w338] -> w313
              tunnel: w312 -> [w335]
              tunnel: [w342] -> w321
              tunnel: w324 -> [w342]
              tunnel: [w341] -> w320
              tunnel: [w340] -> w319
              tunnel: w313 -> [w341]
              frame #0 {
                n103 = call <vilib>:"High Resolution Relative Seconds.vi"() -> ("relative seconds"=w332:dbl)
              }
              frame #1 {
                n104 = call "Write.vim"("error in (no error)"=w339, "Data In"=w336, "Writer Reference"=w335) -> ("error out"=w338:errorcluster, "Data Out"=w337:dbl)  [unwired: 7 in]
              }
              frame #2 {
                n105 = call <vilib>:"High Resolution Relative Seconds.vi"() -> ("relative seconds"=w340:dbl)
              }
            }
            n106 = Subtract(x=w319, y=w318) -> (x-y=w317:dbl)
            n107 = case shown="0" w314 {
              tunnel: w317 -> [_ w330]
              tunnel: w316 -> [w327 w329]
              tunnel: [w327 w328] -> w315
              frame 0 {
              }
              frame 1, Default {
                (unwired) u32 1 ("milliseconds to wait")
                n108 = Max & Min(x=w330, y=w329) -> (max(x,y)=w328:dbl)  [unwired: 1 out]
              }
            }
          }
        }
        "max write double" <- w280
        n109 = while {
          shift-right: [w291] -> w259
          shift-left: w260 -> [w292]
          tunnel: w257 -> [w294]
          stop <- w295 stop-if-true
          n110 = call "Read.vim"("error in (no error)"=w292, "Data In"=3.14 ("Data"), "Reader Reference"=w294) -> ("error out"=w291:errorcluster)  [unwired: 6 in, 2 out]
          n111 = Wait (ms)(milliseconds to wait=u32 10) -> ()  [unwired: 1 out]
          n112 = local read "stop"() -> (w295:bool)
        }
        n113 = node-c288(w289) -> ()  [unwired: 1 out]
        n114 = node-c288(w287) -> ()  [unwired: 1 out]
        n115 = Subtract(x=w286, y=w285) -> (x-y=w284:dbl)
        n116 = flat-sequence {
          tunnel: w277 -> [w300]
          tunnel: [w300] -> w265
          frame #0 {
            n117 = local write "stop"(TRUE ("stop")) -> ()
          }
        }
        n118 = Divide(x=w284, y=w283) -> (x/y=→"avg write double":dbl)
        n119 = Less?(x=w280, y=1e-06) -> (x < y?=w276:bool)
        n120 = call "Destroy Reader.vim"("error in (no error)"=w259, "Reader Reference"=w257) -> ("error out"=w258:errorcluster)  [unwired: 9 in]
        n121 = Merge Errors(w258, w265) -> (w264:errorcluster)
        n122 = call "Destroy Blackboard.vi"("error in (no error)"=w264, "Blackboard Reference"=w273) -> ("error out"=w271:errorcluster)  [unwired: 8 in, 1 out]
      }
      frame 3 {
        w385 = u8[] array[100001 elements] ("U8 Data")
        w390 = "my_blackboard" ("Blackboard name")
        n123 = flat-sequence {
          tunnel: w387 -> [w424]
          tunnel: [w424] -> w386
          frame #0 {
            n124 = local write "stop"(FALSE ("stop")) -> ()
          }
        }
        n125 = Bundle By Name(cluster=T1 {"BlackBoard"="", "Topic"="", "Type Override"=""} ("Topic Full Names"), "BlackBoard"=w390, "Topic"="big_test" ("topic"), "Type Override"="big_array") -> (w391:T1)
        n126 = call "Create Blackboard.vi"("error in (no error)"=w386, "Blackboard name"=w390) -> ("error out"=w401:errorcluster, "Blackboard Reference"=w399:T5)  [unwired: 8 in]
        n127 = call "Create Writer.vim"("error in (no error)"=w401, "Data"=w385, "Topic Name"=w391, "BlackBoard Reference"=w399) -> ("error out"=w400:errorcluster, "Writer Reference"=w396:T6)  [unwired: 5 in, 1 out]
        n128 = call "Start Blackboard.vi"("error in (no error)"=w400, "Blackboard Reference"=w399) -> ("error out"=w398:errorcluster)  [unwired: 9 in]
        n129 = call "Create Reader.vim"("error in (no error)"=w398, "Data Type"=w385, "Topic Name"=w391) -> ("error out"=w395:errorcluster, "Reader Reference"=w381:T7)  [unwired: 6 in, 1 out]
        n130 = call "Read.vim"("error in (no error)"=w395, "Data In"=w385, "Reader Reference"=w381) -> ("error out"=w394:errorcluster)  [unwired: 6 in, 2 out]
        n131 = flat-sequence {
          tunnel: w394 -> [w428]
          tunnel: [w428] -> w404
          frame #0 {
            n132 = Wait (ms)(milliseconds to wait=u32 100) -> ()  [unwired: 1 out]
          }
        }
        n133 = node-c288() -> (w416:T2)
        n134 = node-c288() -> (w414:T2)
        n135 = timed-loop {
          timing: w416 -> [_]
          timing-out: [_] -> w415
          tunnel: w381 -> [w475]
          tunnel: w404 -> [w485]
          tunnel: [w482] -> w408
          tunnel: [w480] -> w412
          tunnel: [w479] -> w411
          tunnel: [w478] -> w409
          tunnel: w385 -> [w473]
          stop <- TRUE stop-if-true
          n136 = flat-sequence {
            tunnel: w485 -> [w489]
            tunnel: [w489] -> w483
            tunnel: [w488] -> w479
            tunnel: [w487] -> w476
            tunnel: w475 -> [w487]
            tunnel: [w486] -> w474
            tunnel: w473 -> [w486]
            tunnel: w483 -> [w494]
            tunnel: [w493] -> w481
            tunnel: [w492] -> w477
            tunnel: w476 -> [w491]
            tunnel: w474 -> [w490]
            tunnel: [w502] -> w482
            tunnel: w481 -> [w502]
            tunnel: [w501] -> w480
            tunnel: [w500] -> w478
            tunnel: w477 -> [w500]
            frame #0 {
              n137 = call <vilib>:"High Resolution Relative Seconds.vi"() -> ("relative seconds"=w488:dbl)
            }
            frame #1 {
              w492 = 1000
              n138 = for {
                N: w492 -> [_]
                shift-right: [w496] -> _
                shift-left: w490 -> [w495]
                shift-right: [w497] -> w493
                shift-left: w494 -> [w498]
                tunnel: w491 -> [w499]
                n139 = call "Read.vim"("error in (no error)"=w498, "Data In"=w495, "Reader Reference"=w499) -> ("error out"=w497:errorcluster, "Data Out"=w496:u8[])  [unwired: 6 in, 1 out]
              }
            }
            frame #2 {
              n140 = call <vilib>:"High Resolution Relative Seconds.vi"() -> ("relative seconds"=w501:dbl)
            }
          }
        }
        n141 = timed-loop {
          timing: w414 -> [_]
          timing-out: [_] -> w413
          tunnel: w408 -> [w436]
          tunnel: [w434] -> w403
          tunnel: [w431] -> w406
          tunnel: w385 -> [w430]
          tunnel: w381 -> [w429]
          stop <- TRUE stop-if-true
          n142 = for {
            N: 1000 -> [_]
            shift-right: [w447] -> _
            shift-left: w430 -> [w449]
            shift-right: [w446] -> w434
            shift-left: w436 -> [w448]
            shift-right: [w441] -> w431
            shift-left: 0.0 -> [w442]
            tunnel: w429 -> [w437]
            i -> [w440]
            n143 = flat-sequence {
              tunnel: w448 -> [w459]
              tunnel: w449 -> [w460]
              tunnel: [w460] -> w452
              tunnel: [w459] -> w451
              tunnel: [w458] -> w444
              tunnel: [w457] -> w438
              tunnel: w437 -> [w457]
              tunnel: w452 -> [w461]
              tunnel: w451 -> [w465]
              tunnel: [w463] -> w450
              tunnel: [w462] -> w439
              tunnel: w438 -> [w464]
              tunnel: [w468] -> w447
              tunnel: w450 -> [w468]
              tunnel: [w467] -> w446
              tunnel: [w466] -> w445
              tunnel: w439 -> [w467]
              frame #0 {
                n144 = call <vilib>:"High Resolution Relative Seconds.vi"() -> ("relative seconds"=w458:dbl)
              }
              frame #1 {
                n145 = call "Read.vim"("error in (no error)"=w465, "Data In"=w461, "Reader Reference"=w464) -> ("error out"=w462:errorcluster, "Data Out"=w463:u8[])  [unwired: 6 in, 1 out]
              }
              frame #2 {
                n146 = call <vilib>:"High Resolution Relative Seconds.vi"() -> ("relative seconds"=w466:dbl)
              }
            }
            n147 = Subtract(x=w445, y=w444) -> (x-y=w443:dbl)
            n148 = case shown="0" w440 {
              tunnel: w443 -> [_ w456]
              tunnel: w442 -> [w453 w455]
              tunnel: [w453 w454] -> w441
              frame 0 {
              }
              frame 1, Default {
                (unwired) u32 1 ("milliseconds to wait")
                n149 = Max & Min(x=w456, y=w455) -> (max(x,y)=w454:dbl)  [unwired: 1 out]
              }
            }
          }
        }
        "max read large array" <- w406
        n150 = while {
          shift-right: [w419] -> w383
          shift-left: w395 -> [w420]
          tunnel: w396 -> [w418]
          tunnel: w385 -> [w417]
          stop <- w421 stop-if-true
          n151 = Wait (ms)(milliseconds to wait=u32 10) -> ()  [unwired: 1 out]
          n152 = call "Write.vim"("error in (no error)"=w420, "Data In"=w417, "Writer Reference"=w418) -> ("error out"=w419:errorcluster)  [unwired: 7 in, 1 out]
          n153 = local read "stop"() -> (w421:bool)
        }
        n154 = node-c288(w415) -> ()  [unwired: 1 out]
        n155 = node-c288(w413) -> ()  [unwired: 1 out]
        n156 = Subtract(x=w412, y=w411) -> (x-y=w410:dbl)
        n157 = flat-sequence {
          tunnel: w403 -> [w426]
          tunnel: [w426] -> w389
          frame #0 {
            n158 = local write "stop"(TRUE ("stop")) -> ()
          }
        }
        n159 = Divide(x=w410, y=w409) -> (x/y=→"avg read large array":dbl)
        n160 = Less?(x=w406, y=3e-05) -> (x < y?=w402:bool)
        n161 = call "Destroy Reader.vim"("error in (no error)"=w383, "Reader Reference"=w381) -> ("error out"=w382:errorcluster)  [unwired: 9 in]
        n162 = Merge Errors(w382, w389) -> (w388:errorcluster)
        n163 = call "Destroy Blackboard.vi"("error in (no error)"=w388, "Blackboard Reference"=w399) -> ("error out"=w397:errorcluster)  [unwired: 8 in, 1 out]
      }
      frame 4 {
        w508 = u8[] array[100001 elements] ("U8 Data")
        w518 = "my_blackboard" ("Blackboard name")
        n164 = flat-sequence {
          tunnel: w515 -> [w550]
          tunnel: [w550] -> w514
          frame #0 {
            n165 = local write "stop"(FALSE ("stop")) -> ()
          }
        }
        n166 = Bundle By Name(cluster=T1 {"BlackBoard"="", "Topic"="", "Type Override"=""} ("Topic Full Names"), "BlackBoard"=w518, "Topic"="big_test2" ("topic"), "Type Override"="big_raw") -> (w519:T1)
        n167 = call "Create Blackboard.vi"("error in (no error)"=w514, "Blackboard name"=w518) -> ("error out"=w527:errorcluster, "Blackboard Reference"=w525:T5)  [unwired: 8 in]
        n168 = call "Create Raw Writer.vi"("error in (no error)"=w527, "Data"=w508, "Topic Name"=w519, "BlackBoard Reference"=w525) -> ("error out"=w526:errorcluster, "Raw Writer Reference"=w522:T8)  [unwired: 5 in, 1 out]
        n169 = call "Start Blackboard.vi"("error in (no error)"=w526, "Blackboard Reference"=w525) -> ("error out"=w524:errorcluster)  [unwired: 9 in]
        n170 = call "Create Raw Reader.vi"("error in (no error)"=w524, "Topic Full Names"=w519) -> ("error out"=w510:errorcluster, "Raw Reader Reference"=w507:T9)  [unwired: 8 in]
        n171 = flat-sequence {
          tunnel: w509 -> [w554]
          tunnel: [w554] -> w530
          frame #0 {
            n172 = Wait (ms)(milliseconds to wait=u32 100) -> ()  [unwired: 1 out]
          }
        }
        n173 = call "Read Raw.vi"("error in (no error)"=w510, "Data In"=w508, "Raw Reader Reference"=w507) -> ("error out"=w509:errorcluster)  [unwired: 5 in, 3 out]
        n174 = node-c288() -> (w542:T2)
        n175 = node-c288() -> (w540:T2)
        n176 = timed-loop {
          timing: w542 -> [_]
          timing-out: [_] -> w541
          tunnel: w507 -> [w601]
          tunnel: w530 -> [w611]
          tunnel: [w608] -> w534
          tunnel: [w606] -> w538
          tunnel: [w605] -> w537
          tunnel: [w604] -> w535
          tunnel: w508 -> [w599]
          stop <- TRUE stop-if-true
          n177 = flat-sequence {
            tunnel: w611 -> [w615]
            tunnel: [w615] -> w609
            tunnel: [w614] -> w605
            tunnel: [w613] -> w602
            tunnel: w601 -> [w613]
            tunnel: [w612] -> w600
            tunnel: w599 -> [w612]
            tunnel: w609 -> [w620]
            tunnel: [w619] -> w607
            tunnel: [w618] -> w603
            tunnel: w602 -> [w617]
            tunnel: w600 -> [w616]
            tunnel: [w628] -> w608
            tunnel: w607 -> [w628]
            tunnel: [w627] -> w606
            tunnel: [w626] -> w604
            tunnel: w603 -> [w626]
            frame #0 {
              n178 = call <vilib>:"High Resolution Relative Seconds.vi"() -> ("relative seconds"=w614:dbl)
            }
            frame #1 {
              w618 = 1000
              n179 = for {
                N: w618 -> [_]
                shift-right: [w622] -> _
                shift-left: w616 -> [w621]
                shift-right: [w623] -> w619
                shift-left: w620 -> [w624]
                tunnel: w617 -> [w625]
                n180 = call "Read Raw.vi"("error in (no error)"=w624, "Data In"=w621, "Raw Reader Reference"=w625) -> ("error out"=w623:errorcluster, "Data Out"=w622:u8[])  [unwired: 5 in, 2 out]
              }
            }
            frame #2 {
              n181 = call <vilib>:"High Resolution Relative Seconds.vi"() -> ("relative seconds"=w627:dbl)
            }
          }
        }
        n182 = timed-loop {
          timing: w540 -> [_]
          timing-out: [_] -> w539
          tunnel: w534 -> [w562]
          tunnel: [w560] -> w529
          tunnel: [w557] -> w532
          tunnel: w508 -> [w556]
          tunnel: w507 -> [w555]
          stop <- TRUE stop-if-true
          n183 = for {
            N: 1000 -> [_]
            shift-right: [w573] -> _
            shift-left: w556 -> [w575]
            shift-right: [w572] -> w560
            shift-left: w562 -> [w574]
            shift-right: [w567] -> w557
            shift-left: 0.0 -> [w568]
            tunnel: w555 -> [w563]
            i -> [w566]
            n184 = flat-sequence {
              tunnel: w574 -> [w585]
              tunnel: w575 -> [w586]
              tunnel: [w586] -> w578
              tunnel: [w585] -> w577
              tunnel: [w584] -> w570
              tunnel: [w583] -> w564
              tunnel: w563 -> [w583]
              tunnel: w578 -> [w587]
              tunnel: w577 -> [w591]
              tunnel: [w589] -> w576
              tunnel: [w588] -> w565
              tunnel: w564 -> [w590]
              tunnel: [w594] -> w573
              tunnel: w576 -> [w594]
              tunnel: [w593] -> w572
              tunnel: [w592] -> w571
              tunnel: w565 -> [w593]
              frame #0 {
                n185 = call <vilib>:"High Resolution Relative Seconds.vi"() -> ("relative seconds"=w584:dbl)
              }
              frame #1 {
                n186 = call "Read Raw.vi"("error in (no error)"=w591, "Data In"=w587, "Raw Reader Reference"=w590) -> ("error out"=w588:errorcluster, "Data Out"=w589:u8[])  [unwired: 5 in, 2 out]
              }
              frame #2 {
                n187 = call <vilib>:"High Resolution Relative Seconds.vi"() -> ("relative seconds"=w592:dbl)
              }
            }
            n188 = Subtract(x=w571, y=w570) -> (x-y=w569:dbl)
            n189 = case shown="0" w566 {
              tunnel: w569 -> [_ w582]
              tunnel: w568 -> [w579 w581]
              tunnel: [w579 w580] -> w567
              frame 0 {
              }
              frame 1, Default {
                (unwired) u32 1 ("milliseconds to wait")
                n190 = Max & Min(x=w582, y=w581) -> (max(x,y)=w580:dbl)  [unwired: 1 out]
              }
            }
          }
        }
        "max read raw large array" <- w532
        n191 = while {
          shift-right: [w545] -> w512
          shift-left: w510 -> [w546]
          tunnel: w522 -> [w544]
          tunnel: w508 -> [w543]
          stop <- w547 stop-if-true
          n192 = Wait (ms)(milliseconds to wait=u32 10) -> ()  [unwired: 1 out]
          n193 = call "Write Raw.vi"("error in (no error)"=w546, "Data In"=w543, "Writer Reference"=w544) -> ("error out"=w545:errorcluster)  [unwired: 7 in, 1 out]
          n194 = local read "stop"() -> (w547:bool)
        }
        n195 = node-c288(w541) -> ()  [unwired: 1 out]
        n196 = node-c288(w539) -> ()  [unwired: 1 out]
        n197 = Subtract(x=w538, y=w537) -> (x-y=w536:dbl)
        n198 = flat-sequence {
          tunnel: w529 -> [w552]
          tunnel: [w552] -> w517
          frame #0 {
            n199 = local write "stop"(TRUE ("stop")) -> ()
          }
        }
        n200 = Divide(x=w536, y=w535) -> (x/y=→"avg read raw large array":dbl)
        n201 = Less?(x=w532, y=2e-05) -> (x < y?=w528:bool)
        n202 = call "Destroy Reader.vim"("error in (no error)"=w512, "Reader Reference"=w507) -> ("error out"=w511:errorcluster)  [unwired: 9 in]
        n203 = Merge Errors(w511, w517) -> (w516:errorcluster)
        n204 = call "Destroy Blackboard.vi"("error in (no error)"=w516, "Blackboard Reference"=w525) -> ("error out"=w523:errorcluster)  [unwired: 8 in, 1 out]
      }
      frame 10, Default {
      }
    }
  }
  n205 = And Array Elements(Boolean array=w2) -> (logical AND=→"pass":bool)
  n206 = call "Shutdown Iceoryx.vi"("error in (no error)"=w6) -> ("error out"=→"error out":errorcluster)  [unwired: 10 in]
